vi "Get Device IDs.vi"() -> ()   [LabVIEW 2021]
uses:
  typedef/Relay ID.ctl
  USB Relay Control.lvlib
panel:
  out "Device List":string[](array[string])
  out "Device IDs":T1[](array[typedef]) {"Serial Number" format="%06x"}
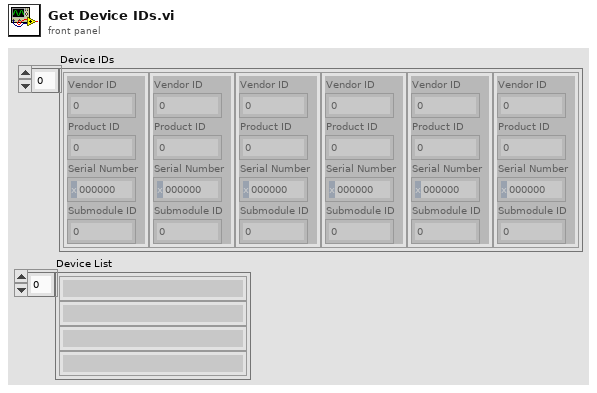
[diagram p1: front panel]
types:
  T1 = typedef "USB Relay Control.lvlib/Relay ID.ctl" = cluster{"Vendor ID":u8, "Product ID":u8, "Serial Number":u32, "Submodule ID":u8}
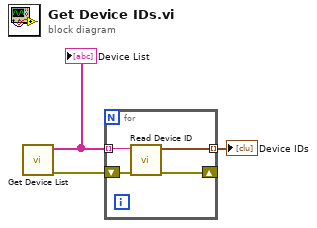
[diagram p0: block diagram]
diagram:
  n1 = call "Get Device List.vi"() -> ("error out"=w2:errorcluster, "Device List"=w3:string[])  [unwired: 10 in]
  "Device List" <- w3
  n2 = for {
    tunnel: w3 -> [w7] mode=indexing
    shift-right: [w5] -> _
    shift-left: w2 -> [w6]
    tunnel: [w4] -> w1 mode=indexing
    n3 = call "Read Device ID.vi"("error in (no error)"=w6, "Device"=w7) -> ("error out"=w5:errorcluster, "Relay ID"=w4:T1)  [unwired: 8 in]
  }
  "Device IDs" <- w1
